vi "EditOptions.vi"(8 "error in":errorcluster, 11 "Engine in":refnum<class "Engine Parent Editor Node.lvclass">) -> (0 "error out":errorcluster, 1 "edit options":T1, 2 "subnodes class":T2, 3 "Engine out":refnum<class "Engine Parent Editor Node.lvclass">)   [LabVIEW 2013, in "PL Framework Configuration Tool.lvlib" / "Engine Parent Editor Node.lvclass"]
doc: "This VI Contains the options for the Menu that will be displayed when doing right click on an item\nThe subnodes class configures which nodes can be added to this nodes\nAnd the edit options determine which options are available for the node.\n\nThis configuration is stored in this VI in case some dynamic configuration is required for the menu options or subnodes.\n\nAll VIs must overide this method"
uses:
  Engine Parent Editor Node.lvclass
  <vilib>/NI/Configuration Framework/Node/SubNodeCluster.ctl
  <vilib>/NI/Configuration Framework/Node/NodeMenuOptions.ctl
  Targets/Targets.lvclass
  subnodes sort by.ctl
  <vilib>/NI/Configuration Framework/Node/NISE_CEF_Node.lvclass/NISE_CEF_Node.ctl
  Targets/Targets.lvclass/Targets.ctl
  Framework Configuration Classes/target configuration/PL_Target Configuration.lvclass/PL_Target Configuration.ctl
  Targets/Read Configuration Class Name.vi
  Framework Configuration Classes/class cache/cache data.vi
  <vilib>/NI/Configuration Framework/Node/NISE_CEF_Node.lvclass
  Framework Configuration Classes/class cache/PL_class cache.lvlib
  Framework Configuration Classes/target configuration/PL_Target Configuration.lvclass
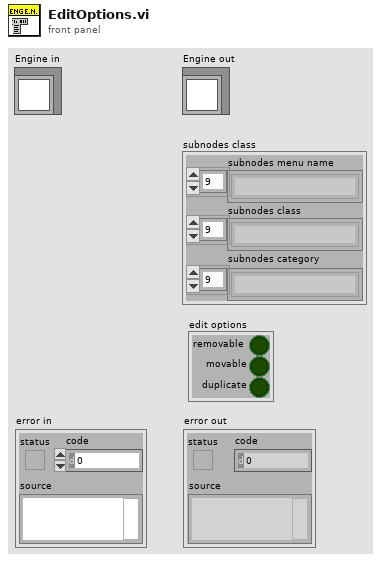
[diagram p1: front panel]
types:
  T1 = typedef "NISE_CEF_Node.lvclass/NodeMenuOptions.ctl" = cluster{"removable":bool, "movable":bool, "duplicate":bool}
  T2 = typedef "NISE_CEF_Node.lvclass/SubNodeCluster.ctl" = cluster{"subnodes menu name":string[], "subnodes class":string[], "subnodes category":string[]}
  T3 = typedef "PL Framework Configuration Tool.lvlib/Engine Parent Editor Node.lvclass/subnodes sort by.ctl" = enum16{"Name", "Class", "Category"}
  T4 = typedef "NISE_CEF_Node.lvclass/NodeRef.ctl" = refnum<data-value>
  T5 = typedef "PL_class cache.lvlib/cached class information.ctl" = cluster{"targets":T6[], "engines":T7[], "modules":T7[], "ignored class list":path[]}
  T6 = typedef "PL_class cache.lvlib/target class metadata.ctl" = cluster{"file name":string, "fully qualified name":string, "menu display name":string, "configuration class name":string}
  T7 = typedef "PL_class cache.lvlib/class metadata.ctl" = cluster{"file name":string, "fully qualified name":string, "menu display name":string, "configuration class":string, "category":string, "instances allowed":i32, "supported targets":T8[]}
  T8 = typedef "TBM configuration.lvclass/Target Types.ctl" = enum16{"Windows", "Mac", "Linux", "Linux RT ARM", "VxWorks", "Pharlap", "Other", "Linux RT x64"}
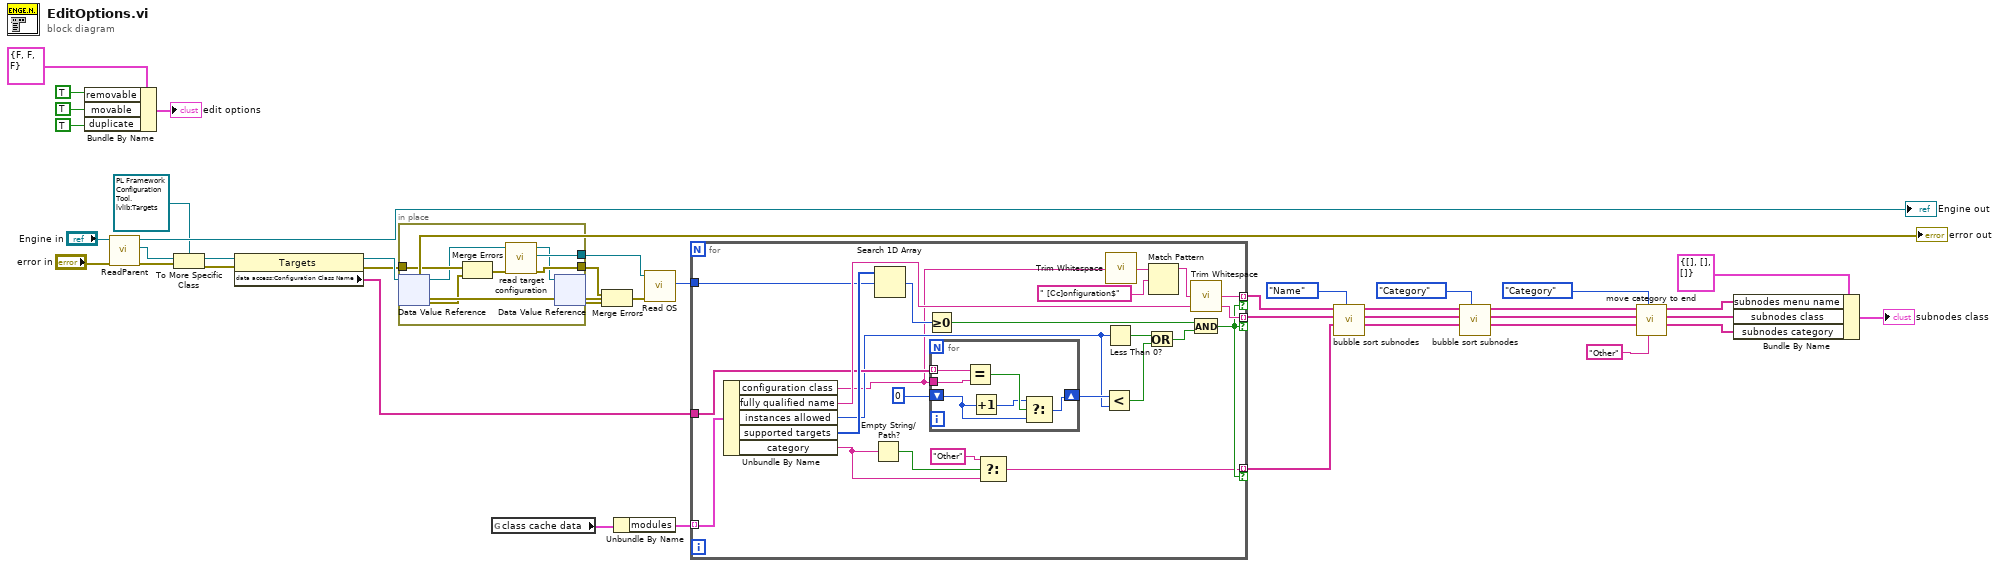
[diagram p0: block diagram]
diagram:
  n1 = Bundle By Name(cluster=T1 {"removable"=FALSE, "movable"=FALSE, "duplicate"=FALSE} ("edit options"), "removable"=TRUE, "movable"=TRUE, "duplicate"=TRUE) -> (→"edit options":T1)
  n2 = call <vilib>:"ReadParent.vi"("error in"="error in", "node in"="Engine in") -> ("error out"=w25:errorcluster, "parent"=w2:T4, "node out"=→"Engine out":refnum<class "Engine Parent Editor Node.lvclass">)  [unwired: 7 in]
  n3 = To More Specific Class(target class=refnum<data-value> refnum, reference=w2, error in=w25) -> (specific class reference=w24:refnum<data-value>, error out=w4:errorcluster)
  n4 = property class="Targets"(reference=w24, error in=w4) -> (reference out=w5:refnum<data-value>, error out=w3:errorcluster, "data access:Configuration Class Name"=w1:string[])
  n5 = in-place {
    in-place-border: [w49] -> w31
    in-place-border: [w48] -> w30
    in-place-border: w3 -> [w47]
    n6 = in-place-dvr #1(w5) -> (w46:refnum<class "Targets.lvclass">, w43:errorcluster)
    n7 = Merge Errors(w47, w43) -> (w44:errorcluster)
    n8 = call "read target configuration.vi"("error in"=w44, "Targets in"=w46) -> ("error out"=w49:errorcluster, "Target Configuration"=w48:refnum<class "PL_Target Configuration.lvclass">, "Targets out"=w45:refnum<class "Targets.lvclass">)  [unwired: 7 in]
    n9 = in-place-dvr #1(w45) -> (w22:errorcluster)  [unwired: 1 out]
  }
  n10 = global read "cache data.vi" "class cache data"() -> (w35:T5)
  n11 = Merge Errors(w31, w22) -> (w23:errorcluster)
  n12 = Unbundle By Name(w35) -> ("modules"=w34:T7[])
  n13 = call "Read OS.vi"("error in"=w23, "PL_Target Configuration in"=w30) -> ("error out"=→"error out":errorcluster, "Target Types"=w29:T8)  [unwired: 7 in, 1 out]
  n14 = for {
    tunnel: w34 -> [w72] mode=indexing
    tunnel: [w55] -> w21 mode=indexing if=w54
    tunnel: [w71] -> w20 mode=indexing if=w54
    tunnel: w1 -> [w67]
    tunnel: w29 -> [w69]
    tunnel: [w50] -> w19 mode=indexing if=w54
    n15 = Unbundle By Name(w72) -> ("configuration class"=w56:string, "fully qualified name"=w71:string, "instances allowed"=w61:i32, "supported targets"=w70:T8[], "category"=w52:string)
    n16 = Empty String/Path?(string/path=w52) -> (empty?=w53:bool)
    n17 = Search 1D Array(1D array=w70, element=w69) -> (index of element=w68:i32)  [unwired: 1 in]
    n18 = Greater Or Equal To 0?(x=w68) -> (x >= 0?=w63:bool)
    n19 = for {
      tunnel: w67 -> [w77] mode=indexing
      tunnel: w56 -> [w78]
      shift-right: [w73] -> w65
      shift-left: 0 -> [w74]
      n20 = Equal?(x=w77, y=w78) -> (x = y?=w76:bool)
      n21 = Increment(x=w74) -> (x+1=w75:i32)
      n22 = Select(t=w75, s=w76, f=w74) -> (s? t:f=w73:i32)
    }
    n23 = Select(t="Other", s=w53, f=w52) -> (s? t:f=w50:string)
    n24 = Less?(x=w65, y=w61) -> (x < y?=w64:bool)
    n25 = Less Than 0?(x=w61) -> (x < 0?=w60:bool)
    n26 = call <vilib>:"Trim Whitespace.vi"("string"=w56) -> ("trimmed string"=w57:string)  [unwired: 1 in]
    n27 = Or(x=w60, y=w64) -> (x .or. y?=w62:bool)
    n28 = Match Pattern(string=w57, regular expression=" [Cc]onfiguration$") -> (before substring=w59:string)  [unwired: 1 in, 3 out]
    n29 = call <vilib>:"Trim Whitespace.vi"("string"=w59) -> ("trimmed string"=w55:string)  [unwired: 1 in]
    n30 = And(x=w63, y=w62) -> (x .and. y?=w54:bool)
  }
  n31 = call "bubble sort subnodes.vi"("Sort by"=subnodes_sort_by."Name", "subnodes category in"=w19, "subnodes class in"=w20, "subnodes menu name in"=w21) -> ("subnodes category out"=w16:string[], "subnodes class out"=w17:string[], "subnodes menu name out"=w18:string[])  [unwired: 5 in]
  n32 = call "bubble sort subnodes.vi"("Sort by"=subnodes_sort_by."Category", "subnodes category in"=w16, "subnodes class in"=w17, "subnodes menu name in"=w18) -> ("subnodes category out"=w13:string[], "subnodes class out"=w14:string[], "subnodes menu name out"=w15:string[])  [unwired: 5 in]
  n33 = call "move category to end.vi"("Category"="Other" ("element"), "Sort by"=subnodes_sort_by."Category", "subnodes category in"=w13, "subnodes class in"=w14, "subnodes menu name in"=w15) -> ("subnodes category out"=w10:string[], "subnodes class out"=w11:string[], "subnodes menu name out"=w12:string[])  [unwired: 4 in]
  n34 = Bundle By Name(cluster=T2 {"subnodes menu name"=[], "subnodes class"=[], "subnodes category"=[]} ("subnodes class"), "subnodes menu name"=w12, "subnodes class"=w11, "subnodes category"=w10) -> (→"subnodes class":T2)
